vi "PicoScope2000aAdvancedTriggerSettings.vi"(0 "error in":errorcluster, 1 "handle in":i16, 3 "Trigger Conditions":T6 {"Condition Logic" items=["AND", "OR", "XOR"]}, 4 "Trigger Delay":u32, 5 "Auto Trigger (ms)":i32, 6 "Channel A Trigger Properties":T3 {"Direction" items=["Above / Inside", "Below / Outside", "Rising / Enter", "Falling / Exit", "Rising or Falling / Enter or Exit", "Above Lower", "Below Lower", "Rising Lower", "Falling Lower", "Positive Runt", "Negative Runt"]; "Threshold Mode" items=["Level", "Window"]}, 7 "Channel D Trigger Properties":T3 {"Direction" items=["Above / Inside", "Below / Outside", "Rising / Enter", "Falling / Exit", "Rising or Falling / Enter or Exit", "Above Lower", "Below Lower", "Rising Lower", "Falling Lower", "Positive Runt", "Negative Runt"]; "Threshold Mode" items=["Level", "Window"]}, 8 "Channel B Trigger Properties":T3 {"Direction" items=["Above / Inside", "Below / Outside", "Rising / Enter", "Falling / Exit", "Rising or Falling / Enter or Exit", "Above Lower", "Below Lower", "Rising Lower", "Falling Lower", "Positive Runt", "Negative Runt"]; "Threshold Mode" items=["Level", "Window"]}, 10 "Digital Port  0":T2 {"Direction Channel 7" items=["Don't Care", "Low", "High", "Rising", "Falling"]; "Direction Channel 6" items=["Don't Care", "Low", "High", "Rising", "Falling"]; "Direction Channel 5" items=["Don't Care", "Low", "High", "Rising", "Falling"]; "Direction Channel 4" items=["Don't Care", "Low", "High", "Rising", "Falling"]; "Direction Channel 3" items=["Don't Care", "Low", "High", "Rising", "Falling"]; "Direction Channel 2" items=["Don't Care", "Low", "High", "Rising", "Falling"]; "Direction Channel 1" items=["Don't Care", "Low", "High", "Rising", "Falling"]; "Direction Channel 0" items=["Don't Care", "Low", "High", "Rising", "Falling"]}, 11 "Ext. Trigger Properties":T3 {"Direction" items=["Above / Inside", "Below / Outside", "Rising / Enter", "Falling / Exit", "Rising or Falling / Enter or Exit", "Above Lower", "Below Lower", "Rising Lower", "Falling Lower", "Positive Runt", "Negative Runt"]; "Threshold Mode" items=["Level", "Window"]}, 12 "Digital Port  1":T1 {"Direction Channel 15" items=["Don't Care", "Low", "High", "Rising", "Falling"]; "Direction Channel 14" items=["Don't Care", "Low", "High", "Rising", "Falling"]; "Direction Channel 13" items=["Don't Care", "Low", "High", "Rising", "Falling"]; "Direction Channel 12" items=["Don't Care", "Low", "High", "Rising", "Falling"]; "Direction Channel 11" items=["Don't Care", "Low", "High", "Rising", "Falling"]; "Direction Channel 10" items=["Don't Care", "Low", "High", "Rising", "Falling"]; "Direction Channel 9" items=["Don't Care", "Low", "High", "Rising", "Falling"]; "Direction Channel 8" items=["Don't Care", "Low", "High", "Rising", "Falling"]}, 13 "Aux. Trigger Properties":T3 {"Direction" items=["Above / Inside", "Below / Outside", "Rising / Enter", "Falling / Exit", "Rising or Falling / Enter or Exit", "Above Lower", "Below Lower", "Rising Lower", "Falling Lower", "Positive Runt", "Negative Runt"]; "Threshold Mode" items=["Level", "Window"]}, 16 "Channel C Trigger Properties":T3 {"Direction" items=["Above / Inside", "Below / Outside", "Rising / Enter", "Falling / Exit", "Rising or Falling / Enter or Exit", "Above Lower", "Below Lower", "Rising Lower", "Falling Lower", "Positive Runt", "Negative Runt"]; "Threshold Mode" items=["Level", "Window"]}, 18 "Pulse Width Qualifier Conditions":T5 {"Condition Logic" items=["AND", "OR", "XOR"]}, 19 "Pulse Width Qualifier Settings":T4 {"Pulse Width Type" items=["None", "Less Than", "Greater Than", "In Range", "Out of Range"]; "Direction" items=["Rising", "Falling"]}) -> (14 "error out":errorcluster, 15 "handle out":i16)   [LabVIEW 2009]
doc: "This VI is an interface for the advanced trigger features of the oscilloscope (a simple trigger can be set using PicoScope3000aSettings.vi, in which case it is not necessary to use this VI)."
uses:
  ps2000a.dll
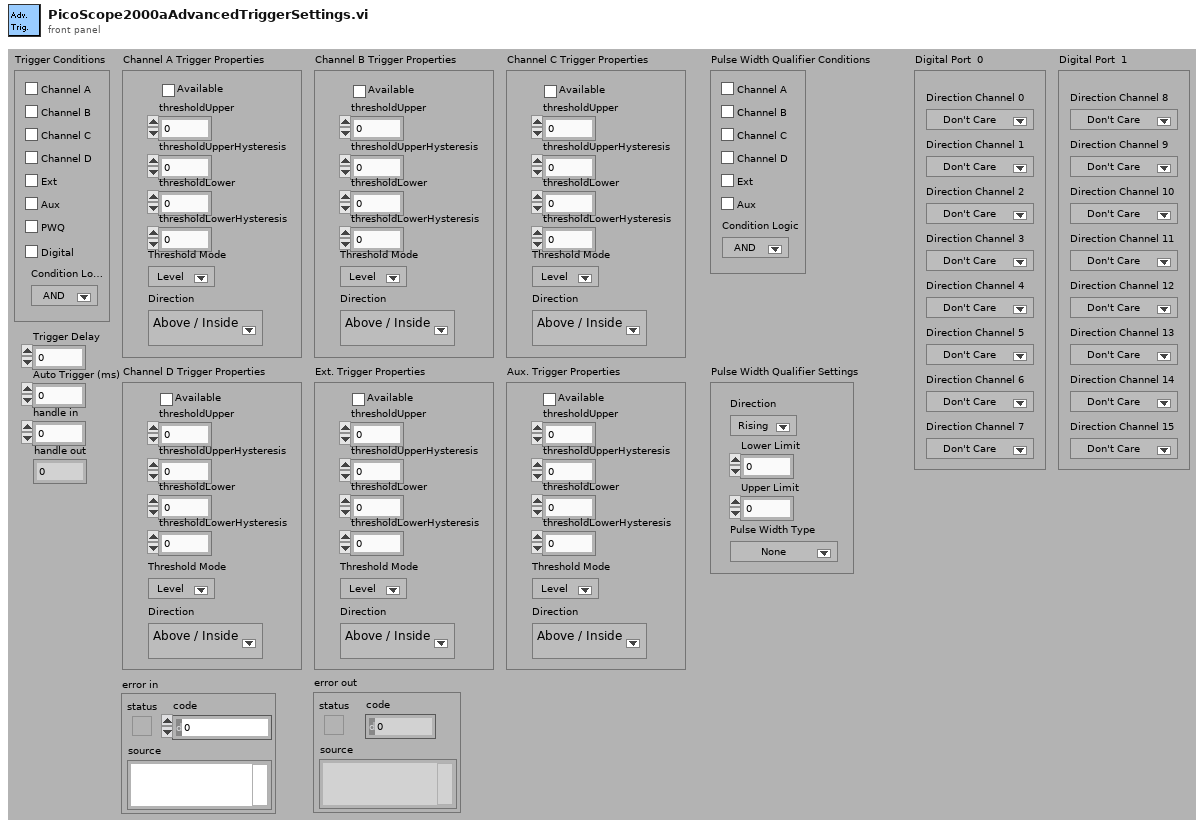
[diagram p1: front panel]
types:
  T1 = cluster{"Direction Channel 8":u16, "Direction Channel 9":u16, "Direction Channel 10":u16, "Direction Channel 11":u16, "Direction Channel 12":u16, "Direction Channel 13":u16, "Direction Channel 14":u16, "Direction Channel 15":u16}
  T2 = cluster{"Direction Channel 0":u16, "Direction Channel 1":u16, "Direction Channel 2":u16, "Direction Channel 3":u16, "Direction Channel 4":u16, "Direction Channel 5":u16, "Direction Channel 6":u16, "Direction Channel 7":u16}
  T3 = cluster{"thresholdUpper":i16, "thresholdUpperHysteresis":u16, "thresholdLower":i16, "thresholdLowerHysteresis":u16, "Threshold Mode":i32, "Direction":i32, "Available":bool}
  T4 = cluster{"Direction":i32, "Lower Limit":u32, "Upper Limit":u32, "Pulse Width Type":i32}
  T5 = cluster{"Channel A":bool, "Channel B":bool, "Channel C":bool, "Channel D":bool, "Aux":bool, "Condition Logic":u16, "Ext":bool}
  T6 = cluster{"Channel A":bool, "Channel B":bool, "Channel C":bool, "Channel D":bool, "Aux":bool, "PWQ":bool, "Condition Logic":u16, "Ext":bool, "Digital":bool}
  T7 = cluster{"thresholdUpper":i16, "thresholdUpperHysteresis":u16, "thresholdLower":i16, "thresholdLowerHysteresis":u16, "Threshold Mode":i32, "Direction":i32, "Available":bool}[]
  T8 = cluster{"[0]":i32, "[1]":i32, "[2]":i32, "[3]":i32, "[4]":i32, "[5]":i32, "[6]":i32, "[7]":i32, "[8]":i32}
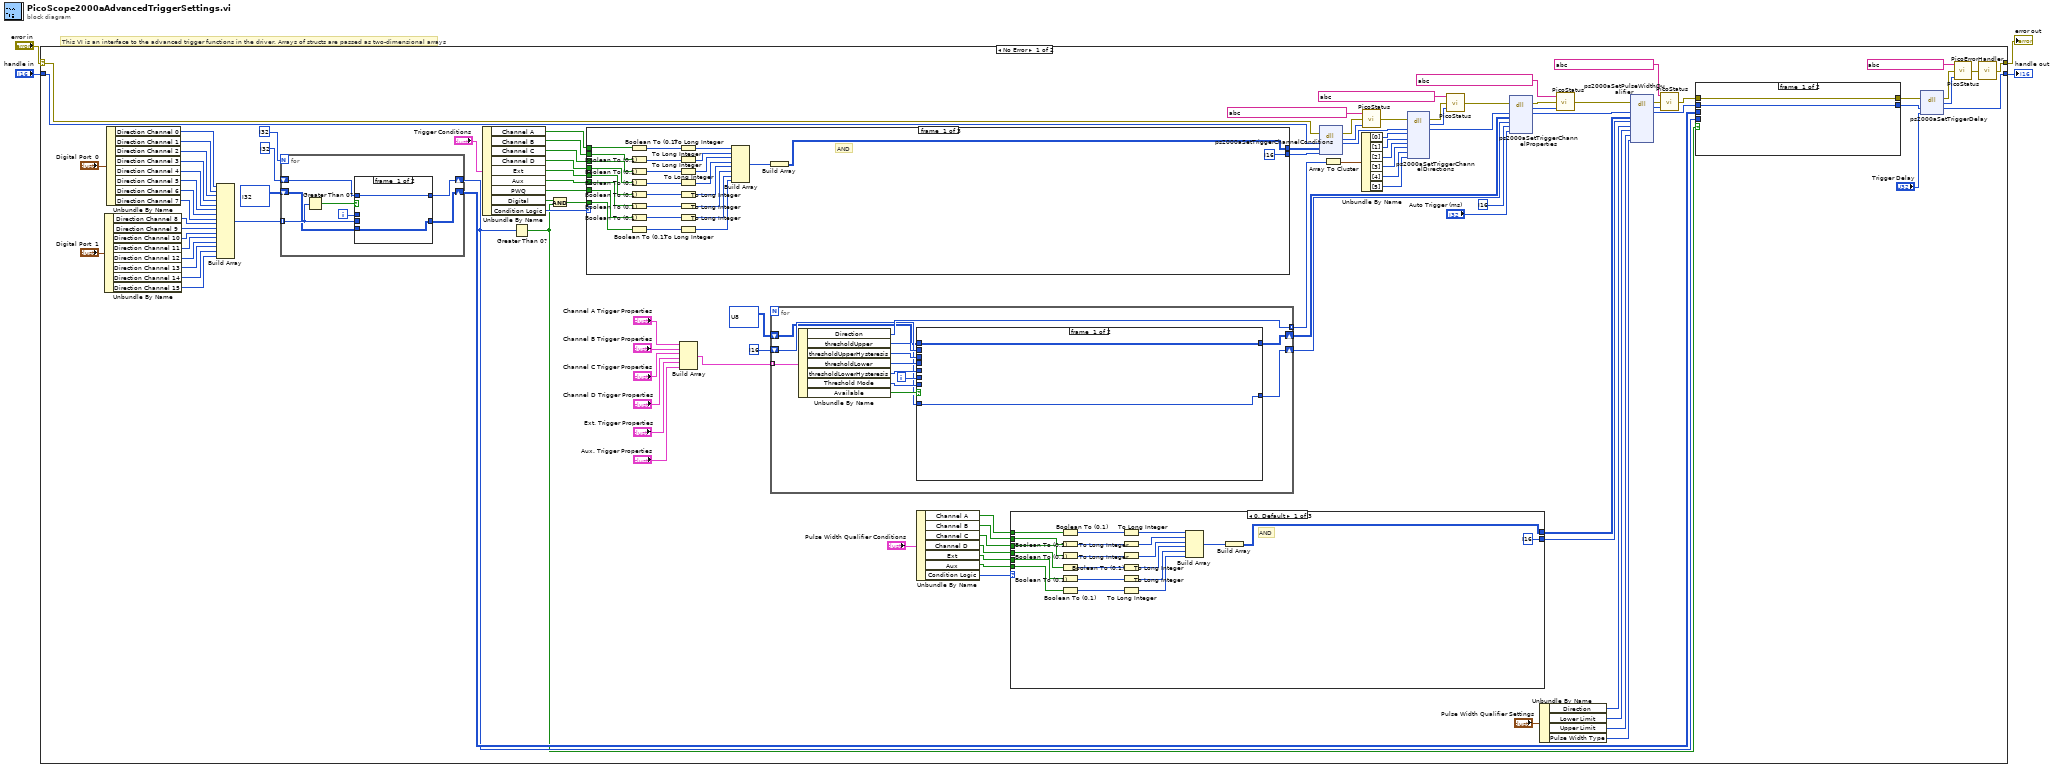
[diagram p0: block diagram]
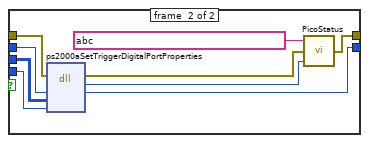
[diagram p2: hidden frame]
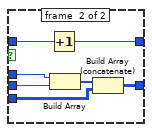
[diagram p3: hidden frame]
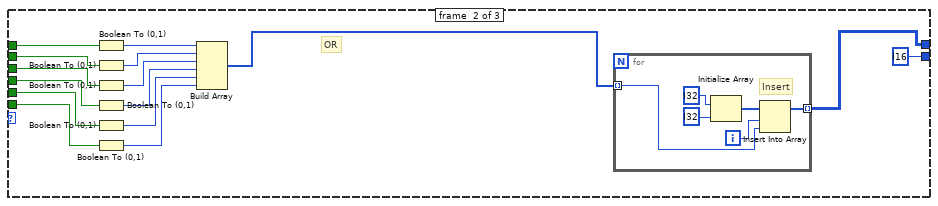
[diagram p4: hidden frame]
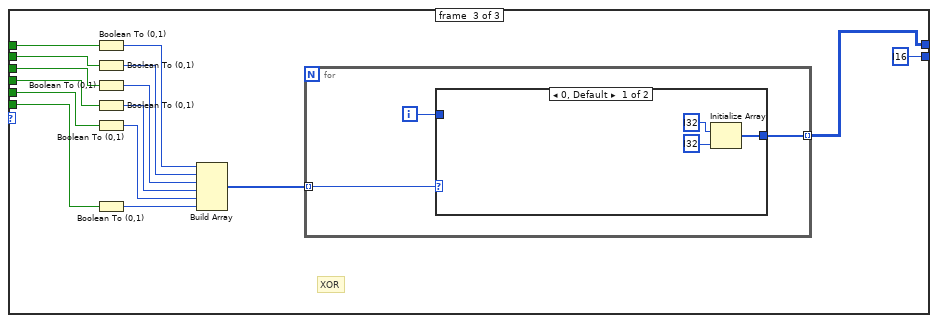
[diagram p5: hidden frame]
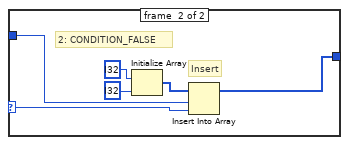
[diagram p6: hidden frame]
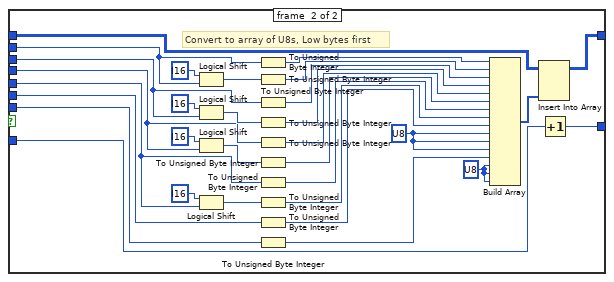
[diagram p7: hidden frame]
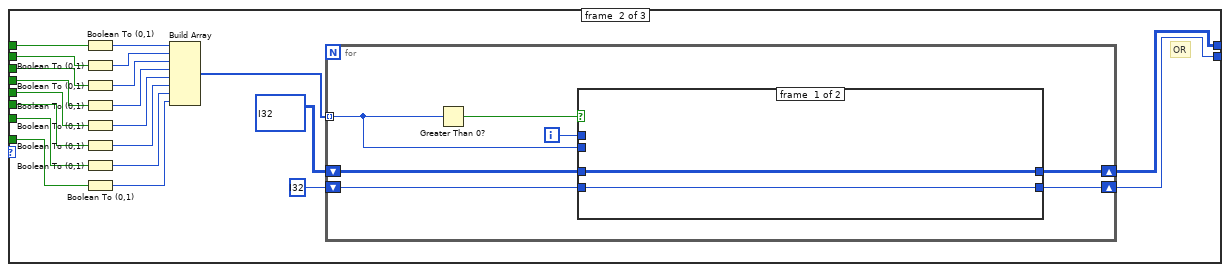
[diagram p8: hidden frame]
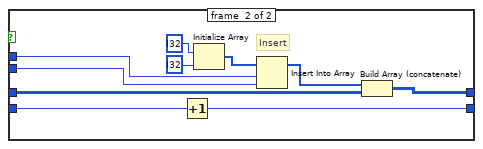
[diagram p9: hidden frame]
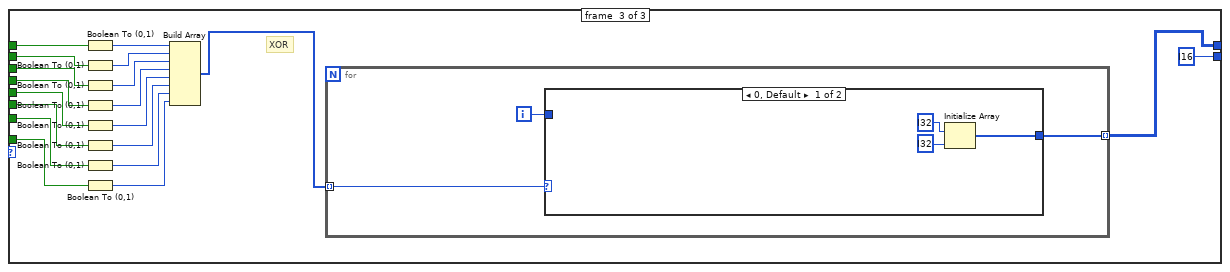
[diagram p10: hidden frame]
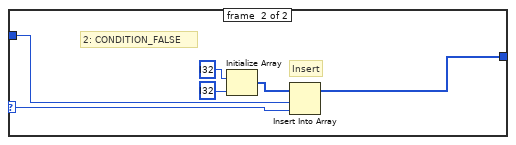
[diagram p11: hidden frame]
diagram:
  # "This VI is an interface to the advanced trigger functions in the driver. Arrays of structs are passed as two-dimensional arrays"
  n1 = case shown="No Error" "error in" {
    selector: "error in" -> [w66 w350]
    tunnel: "handle in" -> [w71 w351]
    tunnel: [w70 w351] -> w2
    tunnel: [w55 w350] -> w1
    frame #0 {
      n2 = Unbundle By Name("Digital Port  1") -> ("Direction Channel 8"=w23:u16, "Direction Channel 9"=w22:u16, "Direction Channel 10"=w21:u16, "Direction Channel 11"=w20:u16, "Direction Channel 12"=w19:u16, "Direction Channel 13"=w18:u16, "Direction Channel 14"=w17:u16, "Direction Channel 15"=w16:u16)
      n3 = Unbundle By Name("Digital Port  0") -> ("Direction Channel 0"=w36:u16, "Direction Channel 1"=w35:u16, "Direction Channel 2"=w34:u16, "Direction Channel 3"=w33:u16, "Direction Channel 4"=w32:u16, "Direction Channel 5"=w31:u16, "Direction Channel 6"=w30:u16, "Direction Channel 7"=w29:u16)
      n4 = Build Array(w36, w35, w34, w33, w32, w31, w30, w29, w23, w22, w21, w20, w19, w18, w17, w16) -> (w26:u16[])
      n5 = for {
        N: i32 ? -> [_]
        tunnel: w26 -> [w125] mode=indexing
        shift-right: [w124] -> w9
        shift-left: i32[][] ? -> [w123]
        shift-right: [w122] -> w6
        shift-left: i32 ? -> [w121]
        i -> [w126]
        n6 = Greater Than 0?(x=w125) -> (x > 0?=w127:bool)
        n7 = case shown="True" w127 {
          tunnel: w126 -> [_ w136]
          tunnel: w125 -> [_ w135]
          tunnel: [w129 w133] -> w124
          tunnel: w123 -> [w129 w132]
          tunnel: [w128 w131] -> w122
          tunnel: w121 -> [w128 w130]
          frame #0 {
          }
          frame #1 {
            n8 = Increment(x=w130) -> (x+1=w131:i32)
            n9 = Build Array(w136, w135) -> (w134:i32[])
            n10 = Build Array (concatenate)(w134, w132) -> (w133:i32[][])
          }
        }
      }
      n11 = Unbundle By Name("Trigger Conditions") -> ("Channel A"=w43:bool, "Channel B"=w42:bool, "Channel C"=w41:bool, "Channel D"=w40:bool, "Ext"=w39:bool, "Aux"=w38:bool, "PWQ"=w37:bool, "Digital"=w8:bool, "Condition Logic"=w44:u16)
      n12 = Greater Than 0?(x=w6) -> (x > 0?=w5:bool)
      n13 = And(x=w8, y=w5) -> (x .and. y?=w7:bool)
      n14 = case shown="1" w44 {
        tunnel: [w263 w291 w329] -> w104
        tunnel: [i16 ? w289 i16 ?] -> w103
        tunnel: w43 -> [w259 w286 w326]
        tunnel: w42 -> [w258 w285 w325]
        tunnel: w41 -> [w257 w284 w324]
        tunnel: w40 -> [w256 w283 w323]
        tunnel: w39 -> [w255 w282 w322]
        tunnel: w38 -> [w254 w281 w321]
        tunnel: w37 -> [w253 w280 w320]
        tunnel: w7 -> [w252 w279 w319]
        frame #0 {
          # "AND"
          n15 = Boolean To (0,1)(Boolean=w259) -> (0, 1=w278:i16)
          n16 = Boolean To (0,1)(Boolean=w258) -> (0, 1=w277:i16)
          n17 = Boolean To (0,1)(Boolean=w257) -> (0, 1=w276:i16)
          n18 = Boolean To (0,1)(Boolean=w256) -> (0, 1=w275:i16)
          n19 = Boolean To (0,1)(Boolean=w255) -> (0, 1=w274:i16)
          n20 = Boolean To (0,1)(Boolean=w254) -> (0, 1=w273:i16)
          n21 = Boolean To (0,1)(Boolean=w253) -> (0, 1=w272:i16)
          n22 = Boolean To (0,1)(Boolean=w252) -> (0, 1=w261:i16)
          n23 = To Long Integer(number=w278) -> (32bit integer=w271:i32)
          n24 = To Long Integer(number=w277) -> (32bit integer=w270:i32)
          n25 = To Long Integer(number=w276) -> (32bit integer=w269:i32)
          n26 = To Long Integer(number=w275) -> (32bit integer=w268:i32)
          n27 = To Long Integer(number=w274) -> (32bit integer=w267:i32)
          n28 = To Long Integer(number=w273) -> (32bit integer=w266:i32)
          n29 = To Long Integer(number=w272) -> (32bit integer=w265:i32)
          n30 = To Long Integer(number=w261) -> (32bit integer=w260:i32)
          n31 = Build Array(w271, w270, w269, w268, w267, w266, w265, w260) -> (w264:i32[])
          n32 = Build Array(w264) -> (w263:i32[][])
        }
        frame #1 {
          # "OR"
          n33 = Boolean To (0,1)(Boolean=w286) -> (0, 1=w293:i16)
          n34 = Boolean To (0,1)(Boolean=w285) -> (0, 1=w294:i16)
          n35 = Boolean To (0,1)(Boolean=w284) -> (0, 1=w295:i16)
          n36 = Boolean To (0,1)(Boolean=w283) -> (0, 1=w296:i16)
          n37 = Boolean To (0,1)(Boolean=w282) -> (0, 1=w297:i16)
          n38 = Boolean To (0,1)(Boolean=w281) -> (0, 1=w298:i16)
          n39 = Boolean To (0,1)(Boolean=w280) -> (0, 1=w299:i16)
          n40 = Boolean To (0,1)(Boolean=w279) -> (0, 1=w287:i16)
          n41 = Build Array(w293, w294, w295, w296, w297, w298, w299, w287) -> (w292:i16[])
          n42 = for {
            tunnel: w292 -> [w303] mode=indexing
            shift-right: [w302] -> w291
            shift-left: i32[][] ? -> [w306]
            shift-right: [w300] -> w289
            shift-left: i32 ? -> [w301]
            i -> [w305]
            n43 = Greater Than 0?(x=w303) -> (x > 0?=w304:bool)
            n44 = case shown="True" w304 {
              tunnel: w306 -> [w308 w311]
              tunnel: w305 -> [_ w315]
              tunnel: w303 -> [_ w314]
              tunnel: [w308 w313] -> w302
              tunnel: w301 -> [w307 w310]
              tunnel: [w307 w309] -> w300
              frame #0 {
              }
              frame #1 {
                # "Insert"
                n45 = Increment(x=w310) -> (x+1=w309:i32)
                n46 = Initialize Array(i32 ? ("element"), i32 ? ("dimension size")) -> (w316:i32[])
                n47 = Insert Into Array(array=w316, index=w315, new element=w314) -> (w312:i32[])
                n48 = Build Array (concatenate)(w312, w311) -> (w313:i32[][])
              }
            }
          }
        }
        frame #2 {
          # "XOR"
          n49 = Boolean To (0,1)(Boolean=w326) -> (0, 1=w331:i16)
          n50 = Boolean To (0,1)(Boolean=w325) -> (0, 1=w332:i16)
          n51 = Boolean To (0,1)(Boolean=w324) -> (0, 1=w333:i16)
          n52 = Boolean To (0,1)(Boolean=w323) -> (0, 1=w334:i16)
          n53 = Boolean To (0,1)(Boolean=w322) -> (0, 1=w335:i16)
          n54 = Boolean To (0,1)(Boolean=w321) -> (0, 1=w336:i16)
          n55 = Boolean To (0,1)(Boolean=w320) -> (0, 1=w337:i16)
          n56 = Boolean To (0,1)(Boolean=w319) -> (0, 1=w327:i16)
          n57 = Build Array(w331, w332, w333, w334, w335, w336, w337, w327) -> (w330:i16[])
          n58 = for {
            tunnel: w330 -> [w338] mode=indexing
            tunnel: [w340] -> w329 mode=indexing
            i -> [w339]
            n59 = case shown="0, Default" w338 {
              selector: w338 -> [_ w345]
              tunnel: [w341 w346] -> w340
              tunnel: w339 -> [_ w344]
              frame #0 {
                n60 = Initialize Array(i32 ? ("element"), i32 ? ("dimension size")) -> (w341:i32[])
              }
              frame #1 {
                # "2: CONDITION_FALSE"
                # "Insert"
                n61 = Initialize Array(i32 ? ("element"), i32 ? ("dimension size")) -> (w347:i32[])
                n62 = Insert Into Array(array=w347, index=w344, new element=w345) -> (w346:i32[])
              }
            }
          }
        }
      }
      n63 = Build Array("Channel A Trigger Properties", "Channel B Trigger Properties", "Channel C Trigger Properties", "Channel D Trigger Properties", "Ext. Trigger Properties", "Aux. Trigger Properties") -> (w101:T7)
      n64 = for {
        tunnel: w101 -> [w213] mode=indexing
        tunnel: [w212] -> w100 mode=indexing
        shift-right: [w209] -> w47
        shift-left: i16 ? -> [w208]
        shift-right: [w206] -> w45
        shift-left: u8[][] ? -> [w207]
        i -> [w210]
        n65 = Unbundle By Name(w213) -> ("Direction"=w212:i32, "thresholdUpper"=w218:i16, "thresholdUpperHysteresis"=w217:u16, "thresholdLower"=w216:i16, "thresholdLowerHysteresis"=w215:u16, "Threshold Mode"=w214:i32, "Available"=w211:bool)
        n66 = case shown="True" w211 {
          tunnel: w218 -> [_ w250]
          tunnel: w217 -> [_ w242]
          tunnel: w216 -> [_ w241]
          tunnel: w215 -> [_ w240]
          tunnel: w214 -> [_ w231]
          tunnel: w210 -> [_ w226]
          tunnel: [w220 w225] -> w209
          tunnel: w208 -> [w220 w224]
          tunnel: [w219 w222] -> w206
          tunnel: w207 -> [w219 w221]
          frame #0 {
          }
          frame #1 {
            w229 = u8 ? ("element")
            w230 = u8 ? ("element")
            # "Convert to array of U8s, Low bytes first"
            n67 = Logical Shift(y=i16 ?, x=w250) -> (x << y=w249:i16)
            n68 = Logical Shift(y=i16 ?, x=w242) -> (x << y=w248:u16)
            n69 = Logical Shift(y=i16 ?, x=w241) -> (x << y=w245:i16)
            n70 = Logical Shift(y=i16 ?, x=w240) -> (x << y=w244:u16)
            n71 = To Unsigned Byte Integer(number=w250) -> (unsigned 8bit integer=w239:u8)
            n72 = To Unsigned Byte Integer(number=w249) -> (unsigned 8bit integer=w238:u8)
            n73 = To Unsigned Byte Integer(number=w242) -> (unsigned 8bit integer=w237:u8)
            n74 = To Unsigned Byte Integer(number=w248) -> (unsigned 8bit integer=w236:u8)
            n75 = To Unsigned Byte Integer(number=w241) -> (unsigned 8bit integer=w235:u8)
            n76 = To Unsigned Byte Integer(number=w245) -> (unsigned 8bit integer=w234:u8)
            n77 = To Unsigned Byte Integer(number=w240) -> (unsigned 8bit integer=w233:u8)
            n78 = To Unsigned Byte Integer(number=w244) -> (unsigned 8bit integer=w232:u8)
            n79 = To Unsigned Byte Integer(number=w226) -> (unsigned 8bit integer=w227:u8)
            n80 = To Unsigned Byte Integer(number=w231) -> (unsigned 8bit integer=w228:u8)
            n81 = Build Array(w239, w238, w237, w236, w235, w234, w233, w232, w227, w230, w230, w230, w228, w229, w229, w229) -> (w223:u8[])
            n82 = Insert Into Array(array=w221, new element=w223) -> (w222:u8[][])  [unwired: 2 in]
            n83 = Increment(x=w224) -> (x+1=w225:i16)
          }
        }
      }
      n84 = Unbundle By Name("Pulse Width Qualifier Conditions") -> ("Channel A"=w90:bool, "Channel B"=w89:bool, "Channel C"=w88:bool, "Channel D"=w87:bool, "Ext"=w86:bool, "Aux"=w77:bool, "Condition Logic"=w78:u16)
      n85 = case shown="0, Default" w78 {
        tunnel: w90 -> [w157 w172 w193]
        tunnel: w89 -> [w151 w171 w192]
        tunnel: w88 -> [w150 w170 w191]
        tunnel: w87 -> [w149 w169 w190]
        tunnel: w86 -> [w148 w160 w181]
        tunnel: [w141 w162 w183] -> w85
        tunnel: [i16 ? i16 ? i16 ?] -> w84
        tunnel: w77 -> [w138 w159 w180]
        frame #0 {
          # "AND"
          n86 = Boolean To (0,1)(Boolean=w157) -> (0, 1=w156:i16)
          n87 = Boolean To (0,1)(Boolean=w151) -> (0, 1=w155:i16)
          n88 = Boolean To (0,1)(Boolean=w150) -> (0, 1=w154:i16)
          n89 = Boolean To (0,1)(Boolean=w149) -> (0, 1=w153:i16)
          n90 = Boolean To (0,1)(Boolean=w148) -> (0, 1=w152:i16)
          n91 = Boolean To (0,1)(Boolean=w138) -> (0, 1=w139:i16)
          n92 = To Long Integer(number=w156) -> (32bit integer=w147:i32)
          n93 = To Long Integer(number=w155) -> (32bit integer=w146:i32)
          n94 = To Long Integer(number=w154) -> (32bit integer=w145:i32)
          n95 = To Long Integer(number=w153) -> (32bit integer=w144:i32)
          n96 = To Long Integer(number=w152) -> (32bit integer=w143:i32)
          n97 = To Long Integer(number=w139) -> (32bit integer=w137:i32)
          n98 = Build Array(w147, w146, w145, w144, w143, w137) -> (w142:i32[])
          n99 = Build Array(w142) -> (w141:i32[][])
        }
        frame #1 {
          # "OR"
          n100 = Boolean To (0,1)(Boolean=w172) -> (0, 1=w164:i16)
          n101 = Boolean To (0,1)(Boolean=w171) -> (0, 1=w165:i16)
          n102 = Boolean To (0,1)(Boolean=w170) -> (0, 1=w166:i16)
          n103 = Boolean To (0,1)(Boolean=w169) -> (0, 1=w167:i16)
          n104 = Boolean To (0,1)(Boolean=w160) -> (0, 1=w168:i16)
          n105 = Boolean To (0,1)(Boolean=w159) -> (0, 1=w158:i16)
          n106 = Build Array(w164, w165, w166, w167, w168, w158) -> (w163:i16[])
          n107 = for {
            tunnel: w163 -> [w174] mode=indexing
            tunnel: [w173] -> w162 mode=indexing
            i -> [w175]
            # "Insert"
            n108 = Initialize Array(i32 ? ("element"), i32 ? ("dimension size")) -> (w176:i32[])
            n109 = Insert Into Array(array=w176, index=w175, new element=w174) -> (w173:i32[])
          }
        }
        frame #2 {
          # "XOR"
          n110 = Boolean To (0,1)(Boolean=w193) -> (0, 1=w185:i16)
          n111 = Boolean To (0,1)(Boolean=w192) -> (0, 1=w186:i16)
          n112 = Boolean To (0,1)(Boolean=w191) -> (0, 1=w187:i16)
          n113 = Boolean To (0,1)(Boolean=w190) -> (0, 1=w188:i16)
          n114 = Boolean To (0,1)(Boolean=w181) -> (0, 1=w189:i16)
          n115 = Boolean To (0,1)(Boolean=w180) -> (0, 1=w179:i16)
          n116 = Build Array(w185, w186, w187, w188, w189, w179) -> (w184:i16[])
          n117 = for {
            tunnel: w184 -> [w196] mode=indexing
            tunnel: [w194] -> w183 mode=indexing
            i -> [w195]
            n118 = case shown="0, Default" w196 {
              selector: w196 -> [_ w201]
              tunnel: [w197 w202] -> w194
              tunnel: w195 -> [_ w200]
              frame #0 {
                n119 = Initialize Array(i32 ? ("element"), i32 ? ("dimension size")) -> (w197:i32[])
              }
              frame #1 {
                # "2: CONDITION_FALSE"
                # "Insert"
                n120 = Initialize Array(i32 ? ("element"), i32 ? ("dimension size")) -> (w203:i32[])
                n121 = Insert Into Array(array=w203, index=w200, new element=w201) -> (w202:i32[])
              }
            }
          }
        }
      }
      n122 = dll-call lib="ps2000a.dll" fn="ps2000aSetTriggerChannelConditions" ("ps3000.dll:_ps3000_open_unit@0")(error in=w66, "handle"=w71, "conditions"=w104, "nConditions"=w103) -> (error out=w68:errorcluster, "PICO_STATUS"=w69:i32, "handle"=w107:i16)  [unwired: 4 in, 1 out]
      n123 = Array To Cluster(array=w100) -> (cluster=w99:T8)
      n124 = Unbundle By Name(w99) -> ("[0]"=w98:i32, "[1]"=w97:i32, "[2]"=w96:i32, "[3]"=w95:i32, "[4]"=w94:i32, "[5]"=w93:i32)
      n125 = call "PicoStatus.vi"("PICO STATUS"=w69, "error in"=w68, "source"=string ?) -> ("error out"=w65:errorcluster)
      n126 = dll-call lib="ps2000a.dll" fn="ps2000aSetTriggerChannelDirections" ("ps3000.dll:_ps3000_open_unit@0")(error in=w65, "handle"=w107, "channelA"=w98, "channelB"=w97, "channelC"=w96, "channelD"=w95, "ext"=w94, "aux"=w93) -> (error out=w63:errorcluster, "PICO_STATUS"=w64:i32, "handle"=w108:i16)  [unwired: 8 in, 1 out]
      n127 = call "PicoStatus.vi"("PICO STATUS"=w64, "error in"=w63, "source"=string ?) -> ("error out"=w54:errorcluster)
      n128 = dll-call lib="ps2000a.dll" fn="ps2000aSetTriggerChannelProperties" ("ps3000.dll:_ps3000_open_unit@0")(error in=w54, "handle"=w108, "channelProperties"=w45, "nChannelProperties"=w47, "auxOutputEnable"=i16 ?, "autoTriggerMilliseconds"="Auto Trigger (ms)") -> (error out=w61:errorcluster, "PICO_STATUS"=w62:i32, "handle"=w106:i16)  [unwired: 6 in, 1 out]
      n129 = Unbundle By Name("Pulse Width Qualifier Settings") -> ("Direction"=w82:i32, "Lower Limit"=w81:u32, "Upper Limit"=w80:u32, "Pulse Width Type"=w79:i32)
      n130 = call "PicoStatus.vi"("PICO STATUS"=w62, "error in"=w61, "source"=string ?) -> ("error out"=w53:errorcluster)
      n131 = dll-call lib="ps2000a.dll" fn="ps2000aSetPulseWidthQualifier" ("ps3000.dll:_ps3000_open_unit@0")(error in=w53, "handle"=w106, "conditions"=w85, "nConditions"=w84, "direction"=w82, "lower"=w81, "upper"=w80, "type"=w79) -> (error out=w59:errorcluster, "PICO_STATUS"=w60:i32, "handle"=w12:i16)  [unwired: 8 in, 1 out]
      n132 = call "PicoStatus.vi"("PICO STATUS"=w60, "error in"=w59, "source"=string ?) -> ("error out"=w13:errorcluster)
      n133 = case shown="True" w5 {
        tunnel: w13 -> [w111 w119]
        tunnel: w12 -> [w110 w118]
        tunnel: [w111 w116] -> w11
        tunnel: [w110 w114] -> w10
        tunnel: w6 -> [_ w113]
        tunnel: w9 -> [_ w112]
        frame #0 {
        }
        frame #1 {
          n134 = dll-call lib="ps2000a.dll" fn="ps2000aSetTriggerDigitalPortProperties"(error in=w119, "handle"=w118, "digitalDirections"=w112, "nDigitalDirections"=w113) -> (error out=w117:errorcluster, "PICO_STATUS"=w115:i32, "handle"=w114:i16)  [unwired: 4 in, 1 out]
          n135 = call "PicoStatus.vi"("PICO STATUS"=w115, "error in"=w117, "source"=string ?) -> ("error out"=w116:errorcluster)
        }
      }
      n136 = dll-call lib="ps2000a.dll" fn="ps2000aSetTriggerDelay" ("ps3000.dll:_ps3000_open_unit@0")(error in=w11, "handle"=w10, "delay"="Trigger Delay") -> (error out=w57:errorcluster, "PICO_STATUS"=w58:i32, "handle"=w70:i16)  [unwired: 3 in, 1 out]
      n137 = call "PicoStatus.vi"("PICO STATUS"=w58, "error in"=w57, "source"=string ?) -> ("error out"=w56:errorcluster)
      n138 = call "PicoErrorHandler.vi"("error in"=w56) -> ("error out"=w55:errorcluster)
    }
    frame #1 {
    }
  }
  "handle out" <- w2
  "error out" <- w1
